vi "Ring CP1252.vi"(0 "Abort Code":u32(ring)=84082688 items=["0503 0000h – Toggle bit not alternated."=84082688, "0504 0001h , comma, here"=84148225, "Größe 5 °C µs"=134217760, "max"=4294967295]) -> (4 "Code Größe":u32)   [LabVIEW 2026]
doc: "Ring repro – Größe"
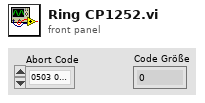
[diagram p1: front panel]
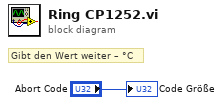
[diagram p0: block diagram]
diagram:
  # "Gibt den Wert weiter – °C"
  "Code Größe" <- "Abort Code"
